vi "Decode Relay ID.vi"(11 "Encoded ID":u8[](array[numeric])=[0, 0, 0, 0, 0] format="%.0x") -> (3 "Relay ID":T1 {"Serial Number" format="%06x"})   [LabVIEW 2021, in "USB Relay Control.lvlib"]
uses:
  USB Relay Control.lvlib
  typedef/Relay ID.ctl
  <vilib>/CIF Foundation/CIF Utilities/DataTypes/Typedef/Endian.ctl
  <vilib>/CIF Foundation/CIF Utilities/DataTypes/DataTypes_CIF_U.lvlib
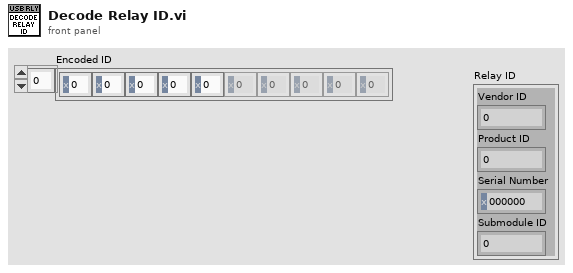
[diagram p1: front panel]
types:
  T1 = typedef "USB Relay Control.lvlib/Relay ID.ctl" = cluster{"Vendor ID":u8, "Product ID":u8, "Serial Number":u32, "Submodule ID":u8}
  T2 = typedef "DataTypes_CIF_U.lvlib/Endian.ctl" = enum16{"Little Endian", "Big Endian"}
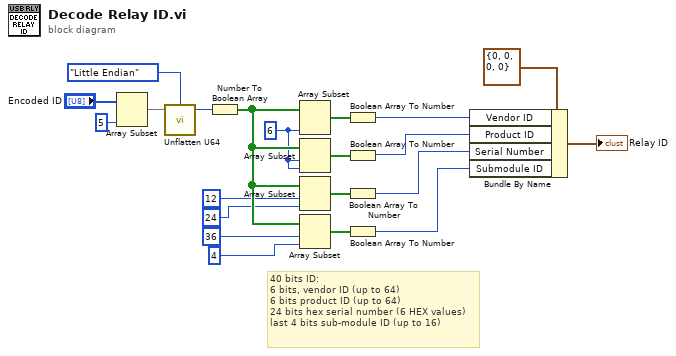
[diagram p0: block diagram]
diagram:
  w18 = 6 ("length")
  # "40 bits ID:\n6 bits, vendor ID (up to 64)\n6 bits product ID (up to 64)\n24 bits hex serial number (6 HEX values)\nlast 4 bits sub-module ID (up to 16)"
  n1 = Array Subset(array="Encoded ID", length=5) -> (w1:u8[])  [unwired: 1 in]
  n2 = call <vilib>:"Unflatten U64.vi"("Flat Data"=w1, "Endian"=Endian."Little Endian") -> ("U64"=w20:u64)  [unwired: 3 in]
  n3 = Number To Boolean Array(number=w20) -> (Boolean array=w19:bool[])
  n4 = Array Subset(array=w19, length=w18) -> (w13:bool[])  [unwired: 1 in]
  n5 = Array Subset(array=w19, index=w18, length=w18) -> (w12:bool[])
  n6 = Array Subset(array=w19, index=12, length=24) -> (w10:bool[])
  n7 = Array Subset(array=w19, index=36, length=4) -> (w11:bool[])
  n8 = Boolean Array To Number(Boolean array=w13) -> (number=w7:u8)
  n9 = Boolean Array To Number(Boolean array=w12) -> (number=w6:u8)
  n10 = Boolean Array To Number(Boolean array=w10) -> (number=w5:u32)
  n11 = Boolean Array To Number(Boolean array=w11) -> (number=w4:u8)
  n12 = Bundle By Name(cluster=T1 {"Vendor ID"=0, "Product ID"=0, "Serial Number"=0, "Submodule ID"=0} ("Relay ID"), "Vendor ID"=w7, "Product ID"=w6, "Serial Number"=w5, "Submodule ID"=w4) -> (→"Relay ID":T1)
